vi "List Channels.vi"(8 "error in (no error)":errorcluster, 11 "E2E editor node in":refnum<data-value>) -> (0 "error out":errorcluster, 1 "Output Channels":refnum<class "TBM channel.lvclass">[](array[class]), 2 "Input Channels":refnum<class "TBM channel.lvclass">[](array[class]), 3 "E2E editor node out":refnum<data-value>)   [LabVIEW 2015, in "E2E Tag Exchange editor node.lvclass"]
uses:
  E2E Tag Exchange editor node.lvclass
  <vilib>/NI/Tag Bus Module Framework/channel/TBM channel.lvclass
  E2E Tag Exchange editor node.lvclass/E2E Tag Exchange editor node.ctl
  module/configuration/E2E Tag Exchange configuration.lvclass
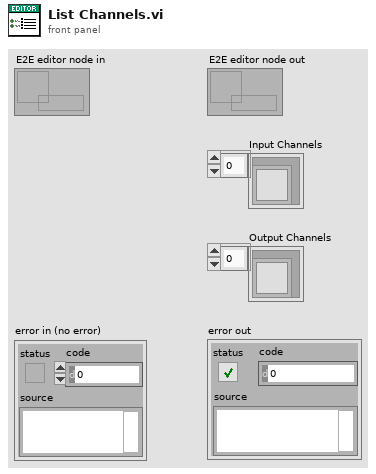
[diagram p1: front panel]
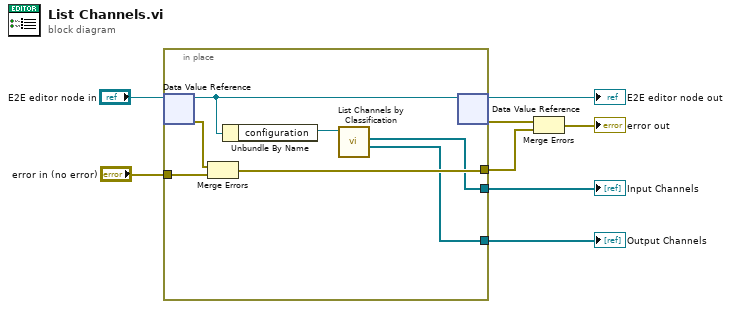
[diagram p0: block diagram]
diagram:
  n1 = in-place {
    in-place-border: "error in (no error)" -> [w13]
    in-place-border: [w11] -> w5
    in-place-border: [w10] -> w2
    in-place-border: [w9] -> w1
    n2 = in-place-dvr #1("E2E editor node in") -> (w15:refnum<class "E2E Tag Exchange editor node.lvclass">, w14:errorcluster)
    n3 = Merge Errors(w14, w13) -> (w11:errorcluster)
    n4 = Unbundle By Name(w15) -> ("configuration"=w12:refnum<class "E2E Tag Exchange configuration.lvclass">)
    n5 = call "List Channels by Classification.vi"("E2E configuration in"=w12) -> ("Output Channels"=w9:refnum<class "TBM channel.lvclass">[], "Input Channels"=w10:refnum<class "TBM channel.lvclass">[])  [unwired: 8 in, 1 out]
    n6 = in-place-dvr #1(w15) -> (→"E2E editor node out":refnum<data-value>, w6:errorcluster)
  }
  "Input Channels" <- w2
  "Output Channels" <- w1
  n7 = Merge Errors(w6, w5) -> (→"error out":errorcluster)
